vi "RemoteVI Capture Window.vi"(0 "hwnd":u64, 11 "error in":errorcluster) -> (4 "pixmap":u32[][](array[numeric]), 6 "rect":cluster{"x":i32, "y":i32, "w":i32, "h":i32}, 15 "error out":errorcluster)   [LabVIEW 2020, in "RemoteVI.lvlib"]
doc: "Captures the window hwnd into a 2D U32 pixmap [row, column] of 0x00RRGGBB values by asking the window to draw itself (user32 PrintWindow with flags 0 - the window paints itself through WM_PRINT; PW_RENDERFULLCONTENT 2 gave the same pixels for the panel and for LabVIEW's menus, colour picker and line width popup but took 2 to 8 times as long, 35 instead of 16 ms for an 837 x 586 panel and 38 instead of 5 ms for the plot legend menu, measured on LabVIEW 2025) into a memory bitmap - GetWindowRect for the size, GetDC(0), CreateCompatibleDC, CreateCompatibleBitmap, SelectObject, PrintWindow, GetDIBits as 32-bit top-down rows. Unlike a screen copy this sees the window's own pixels whether or not it is covered, on another monitor or made invisible (layered with alpha 0, RemoteVI Hide Window.vi) - measured on LabVIEW's popup menus (LVMenuWnd). No VI Server call, so it works while an open popup blocks LabVIEW's UI thread. Every GDI object is deselected and released again, also when an earlier step failed. error out carries error in, a Call Library Function Node error, 5002 when PrintWindow failed or 5001 when GetDIBits copied no line (the window is gone or empty); pixmap may then be all zero or empty."
uses:
  RemoteVI.lvlib
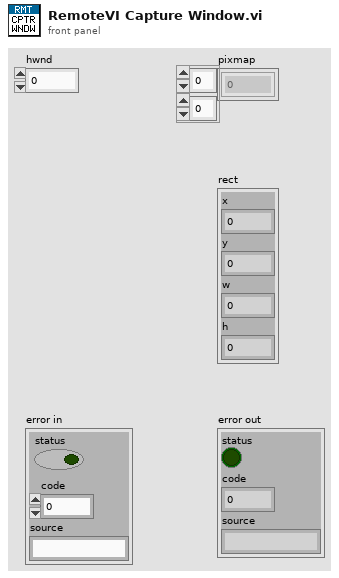
[diagram p1: front panel]
types:
  T1 = cluster{"left":i32, "top":i32, "right":i32, "bottom":i32}
  T2 = cluster{"biSize":u32, i32, i32, "biPlanes":u16, "biBitCount":u16, u32, u32, "zero":i32, "zero":i32, u32, u32, u32}
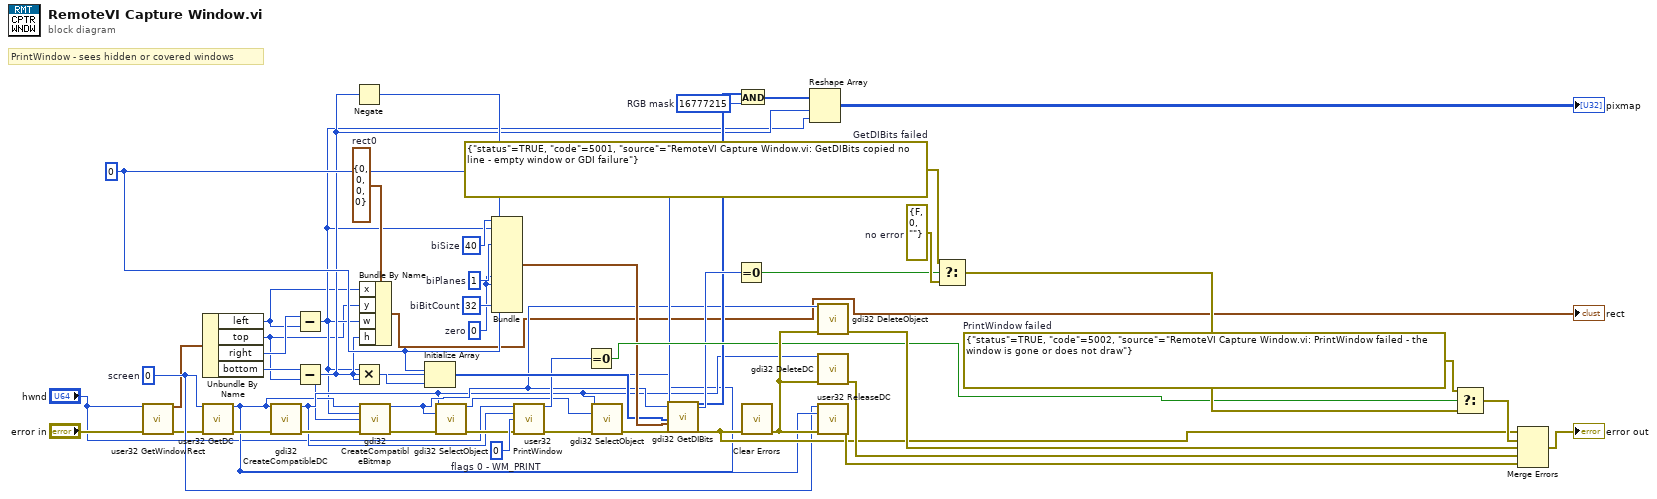
[diagram p0: block diagram]
diagram:
  w46 = errorcluster {"status"=FALSE, "code"=0, "source"=""}  # no error
  w45 = errorcluster {"status"=TRUE, "code"=5001, "source"="RemoteVI Capture Window.vi: GetDIBits copied no line - empty window or GDI failure"}  # GetDIBits failed
  w44 = errorcluster {"status"=TRUE, "code"=5002, "source"="RemoteVI Capture Window.vi: PrintWindow failed - the window is gone or does not draw"}  # PrintWindow failed
  w40 = u32 16777215  # RGB mask
  w35 = u16 32  # biBitCount
  w34 = u16 1  # biPlanes
  w33 = u32 40  # biSize
  w30 = 0  # zero
  w29 = u32 0
  w24 = u32 0  # flags 0 - WM_PRINT
  w15 = u64 0  # screen
  w14 = cluster{"x":i32, "y":i32, "w":i32, "h":i32} {"x"=0, "y"=0, "w"=0, "h"=0}  # rect0
  # "PrintWindow - sees hidden or covered windows"
  n1 = call "user32 GetWindowRect.vi"("hWnd"="hwnd", "error in"="error in") -> ("RECT"=w6:T1, "error out"=w7:errorcluster)  [unwired: 11 in, 1 out]
  n2 = Unbundle By Name(w6) -> ("left"=w8:i32, "top"=w9:i32, "right"=w10:i32, "bottom"=w11:i32)
  n3 = call "user32 GetDC.vi"("hWnd"=w15, "error in"=w7) -> ("HDC"=w16:u64, "error out"=w17:errorcluster)  [unwired: 12 in]
  n4 = call "gdi32 CreateCompatibleDC.vi"("hdc"=w16, "error in"=w17) -> ("HDC"=w18:u64, "error out"=w19:errorcluster)  [unwired: 12 in]
  n5 = Subtract(x=w10, y=w8) -> (x-y=w12:i32)
  n6 = Subtract(x=w11, y=w9) -> (x-y=w13:i32)
  n7 = Negate(x=w13) -> (-x=w32:i32)
  n8 = Multiply(x=w12, y=w13) -> (x*y=w28:i32)
  n9 = Bundle By Name(cluster=w14, "x"=w8, "y"=w9, "w"=w12, "h"=w13) -> (→"rect":cluster{"x":i32, "y":i32, "w":i32, "h":i32})
  n10 = call "gdi32 CreateCompatibleBitmap.vi"("hdc"=w16, "cx"=w12, "cy"=w13, "error in"=w19) -> ("HBITMAP"=w20:u64, "error out"=w21:errorcluster)  [unwired: 10 in]
  n11 = Initialize Array(w29, w28) -> (w31:u32[])
  n12 = call "gdi32 SelectObject.vi"("hdc"=w18, "h"=w20, "error in"=w21) -> ("previous object"=w22:u64, "error out"=w23:errorcluster)  [unwired: 11 in]
  n13 = Bundle("biSize"=w33, w12, w32, "biPlanes"=w34, "biBitCount"=w35, w29, w29, "zero"=w30, "zero"=w30, w29, w29, w29) -> (w36:T2)  [unwired: 1 in]
  n14 = call "user32 PrintWindow.vi"("hwnd"="hwnd", "hdcBlt"=w18, "nFlags"=w24, "error in"=w23) -> ("return value"=w25:i32, "error out"=w26:errorcluster)  [unwired: 10 in]
  n15 = Equal To 0?(x=w25) -> (x = 0?=w42:bool)
  n16 = call "gdi32 SelectObject.vi"("hdc"=w18, "h"=w22, "error in"=w26) -> ("error out"=w27:errorcluster)  [unwired: 11 in, 1 out]
  n17 = call "gdi32 GetDIBits.vi"("hdc"=w16, "hbm"=w20, "start"=w29, "cLines"=w13, "lpvBits"=w31, "lpbmi"=w36, "usage"=w29, "error in"=w27) -> ("lpvBits out"=w37:u32[], "return value"=w38:i32, "error out"=w39:errorcluster)  [unwired: 17 in]
  n18 = Equal To 0?(x=w38) -> (x = 0?=w43:bool)
  n19 = And(x=w37, y=w40) -> (x .and. y?=w41:u32[])
  n20 = call <vilib>:"Clear Errors.vi"("error in (no error)"=w39) -> ("error out"=w49:errorcluster)  [unwired: 5 in, 1 out]
  n21 = Reshape Array(w41, w13, w12) -> (→"pixmap":u32[][])
  n22 = call "gdi32 DeleteObject.vi"("ho"=w20, "error in"=w49) -> ("error out"=w50:errorcluster)  [unwired: 12 in, 1 out]
  n23 = call "gdi32 DeleteDC.vi"("hdc"=w18, "error in"=w49) -> ("error out"=w51:errorcluster)  [unwired: 12 in, 1 out]
  n24 = call "user32 ReleaseDC.vi"("hWnd"=w15, "hDC"=w16, "error in"=w49) -> ("error out"=w52:errorcluster)  [unwired: 11 in, 1 out]
  n25 = Select(t=w45, s=w43, f=w46) -> (s? t:f=w47:errorcluster)
  n26 = Select(t=w44, s=w42, f=w47) -> (s? t:f=w48:errorcluster)
  n27 = Merge Errors(w39, w48, w50, w51, w52) -> (→"error out":errorcluster)
